vi "FlatToRichauth_SubscribeLoginRequest.vi"(5 "OutputClusterType":T1, 11 "InputCluster":T2) -> (3 "OutputCluster":T1)   [LabVIEW 2020, in "grpc-auth_client.lvlib"]
uses:
  auth_SubscribeLoginRequest_Flat.ctl
  auth_SubscribeLoginRequest.ctl
  grpc-auth_client.lvlib
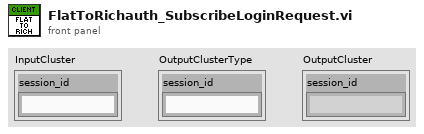
[diagram p1: front panel]
types:
  T1 = typedef "grpc-auth_client.lvlib/auth_SubscribeLoginRequest.ctl" = cluster{"session_id":string}
  T2 = typedef "grpc-auth_client.lvlib/auth_SubscribeLoginRequest_Flat.ctl" = cluster{"session_id":string}
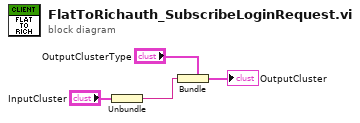
[diagram p0: block diagram]
diagram:
  n1 = Unbundle "Unbundle"("InputCluster") -> ("session_id"=w1:string)
  n2 = Bundle "Bundle"(cluster="OutputClusterType", "session_id"=w1) -> (→"OutputCluster":T1)
